vi "WIFI_Cred.vi"(8 "error in":errorcluster) -> (0 "error out":errorcluster, 1 "Command Response":string, 2 "Result":string, 3 "RESULT":bool)   [LabVIEW 2021]
uses:
  10054_Control Folder/Support/Relay_no.ctl
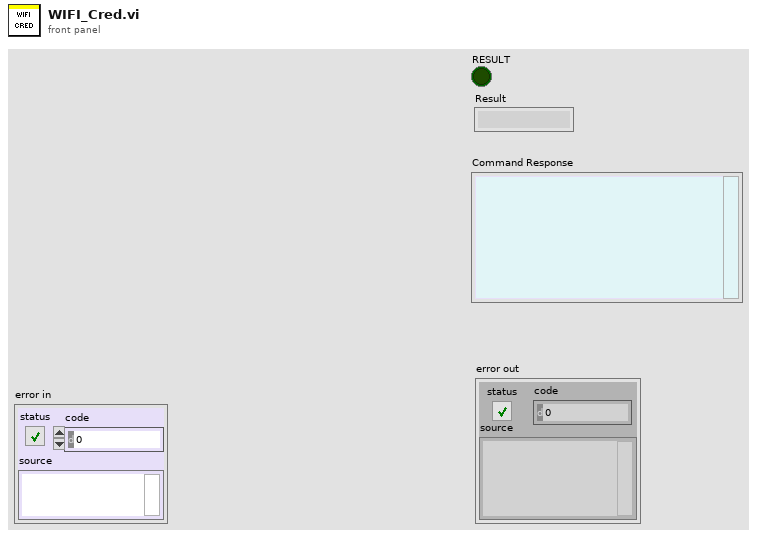
[diagram p1: front panel]
types:
  T1 = typedef "Relay_no.ctl" = enum16{"Init", "write&Read", "PCB Serial Write & Read", "PCB Write SSD & Password", "Read Wifi state", "Reset", "Close"}
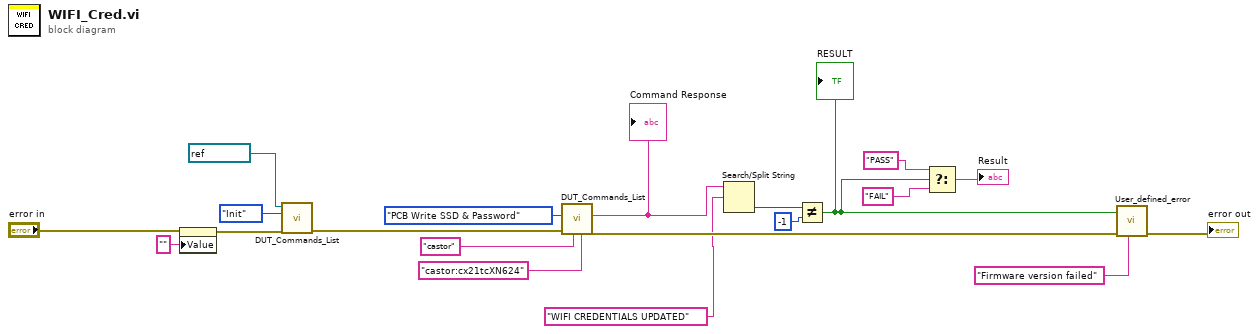
[diagram p0: block diagram]
diagram:
  n1 = property on="Command Response" class="Str"(error in="error in", "Value"="" ("Command Response")) -> (error out=w5:errorcluster)  [unwired: 1 in, 1 out]
  n2 = call "DUT_Commands_List.vi"("error in"=w5, "Operation"=Relay_no."Init", "Resource In"=refnum<visa-resource-name> "COM3") -> ("error out"=w4:errorcluster)  [unwired: 6 in, 2 out]
  n3 = call "DUT_Commands_List.vi"("Password"="castor:cx21tcXN624", "SSID"="castor", "error in"=w4, "Operation"=Relay_no."PCB Write SSD & Password") -> ("error out"=w7:errorcluster, "Command Response"=w12:string)  [unwired: 5 in, 1 out]
  "Command Response" <- w12
  n4 = Search/Split String(string=w12, search string/char (-)="WIFI CREDENTIALS UPDATED") -> (offset of match=w19:i32)  [unwired: 1 in, 2 out]
  n5 = Not Equal?(x=w19, y=-1) -> (x != y?=w16:bool)
  "RESULT" <- w16
  n6 = Select(t="PASS", s=w16, f="FAIL") -> (s? t:f=→"Result":string)
  n7 = call "User_defined_error.vi"("Error Msg"="Firmware version failed" ("source"), "error in"=w7, "Result"=w16) -> ("error Out"=→"error out":errorcluster)  [unwired: 8 in]
